vi "Test Write and Read.vi"(8 "error in (no error)":errorcluster) -> (0 "error out":errorcluster)   [LabVIEW 2020]
doc: "Test case to validate reading from and writing to the dictionary."
uses:
  Classes/Integer Dictionary.lvclass
  classes/Test/Test.lvclass
  classes/Assert/Assert.lvclass
panel:
  # "See block diagram"
  # "Run this VI to execute the unit test. The unit test intentionally fails."
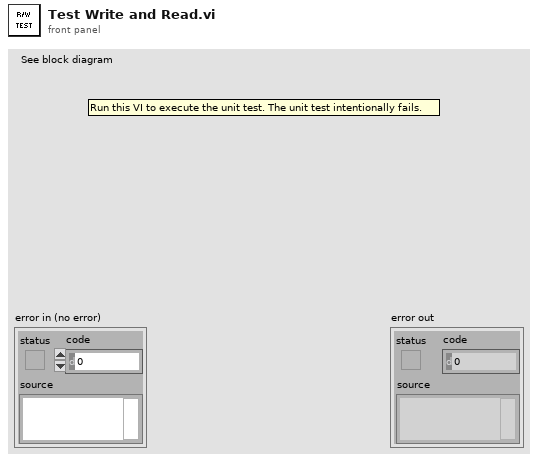
[diagram p1: front panel]
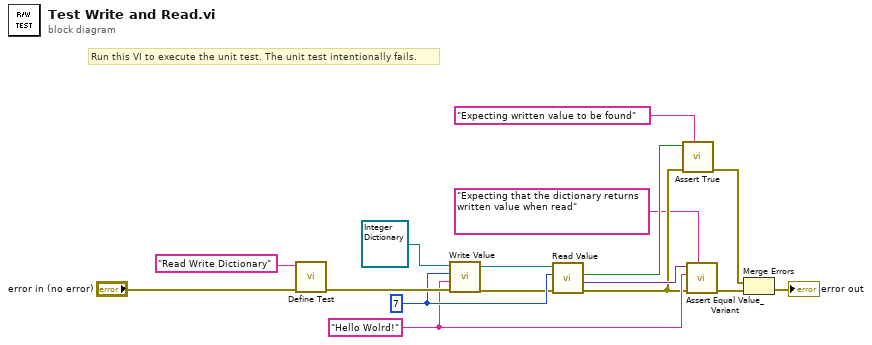
[diagram p0: block diagram]
diagram:
  w4 = "Hello Wolrd!"
  w11 = 7 ("Key")
  # "Run this VI to execute the unit test. The unit test intentionally fails."
  n1 = call "Define Test.vi"("error in (no error)"="error in (no error)", "Label (VI Title)"="Read Write Dictionary") -> ("error out"=w13:errorcluster)  [unwired: 8 in, 1 out]
  n2 = call "Write Value.vi"("error in (no error)"=w13, "Value"=w4, "Key"=w11, "Integer Dictionary in"=refnum<class "Integer Dictionary.lvclass"> refnum) -> ("error out"=w10:errorcluster, "Integer Dictionary out"=w12:refnum<class "Integer Dictionary.lvclass">)  [unwired: 5 in, 1 out]
  n3 = call "Read Value.vi"("error in (no error)"=w10, "Key"=w11, "Integer Dictionary in"=w12) -> ("error out"=w3:errorcluster, "Value"=w5:variant, "found?"=w9:bool)  [unwired: 5 in, 1 out]
  n4 = call "Assert True.vi"("Label"="Expecting written value to be found", "error in (no error)"=w3, "True?"=w9) -> ("error out"=w7:errorcluster)  [unwired: 7 in, 1 out]
  n5 = call "Assert Equal Value_Variant.vi"("Label"="Expecting that the dictionary returns written value when read", "error in (no error)"=w3, "Y"=w4, "X"=w5) -> ("error out"=w2:errorcluster)  [unwired: 6 in, 1 out]
  n6 = Merge Errors(w7, w2) -> (→"error out":errorcluster)
